vi "Tutorial.vi"() -> ()   [LabVIEW 2026]
uses:
  C:/Users/loicw/Documents/LabVIEW/ToastNotifications/Sources/bins/Microsoft.Toolkit.Uwp.Notifications.dll
  bins/Microsoft.Toolkit.Uwp.Notifications.dll
panel:
  out "GetContent":string
  out "Arguments":string
  out "WasCurrentProcessToastActivated":bool
  in  "stop":bool
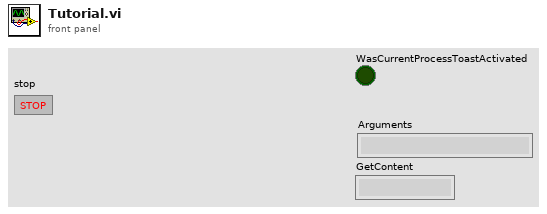
[diagram p1: front panel]
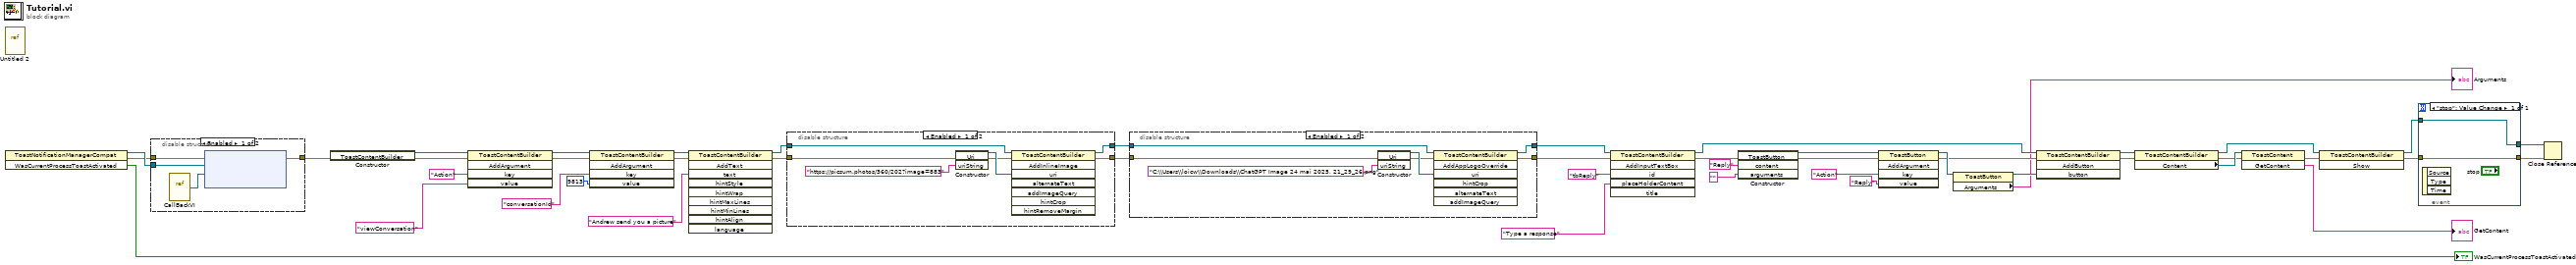
[diagram p0: block diagram]
diagram:
  n1 = vi-ref "Untitled 2.vi"() -> ()  [unwired: 1 out]
  n2 = invoke class="ToastNotificationManagerCompat" method="WasCurrentProcessToastActivated"() -> (reference out=w17:refnum<k24>, error out=w16:errorcluster, "WasCurrentProcessToastActivated"=→"WasCurrentProcessToastActivated":bool)  [unwired: 3 in]
  n3 = disable-structure shown="Enabled" {
    disable-tunnel: w17 -> [w50 _]
    disable-tunnel: w16 -> [w49 w51]
    disable-tunnel: [w48 w51] -> w15
    frame Enabled {
      n4 = vi-ref "CallBackVI.vi"() -> ("vi reference"=w47:refnum<vi>)
      n5 = node(w49, w50, w47) -> (w48:errorcluster)  [unwired: 2 in, 1 out]
    }
    frame Disabled {
    }
  }
  n6 = constructor class="ToastContentBuilder"(error in=w15) -> (reference out=w45:refnum<k24>, error out=w46:errorcluster)  [unwired: 2 in, 1 out]
  n7 = invoke class="ToastContentBuilder" method="AddArgument"(reference=w45, error in=w46, "key"="Action", "value"="viewConversation") -> (reference out=w42:refnum<k24>, error out=w41:errorcluster)  [unwired: 1 in, 3 out]
  n8 = invoke class="ToastContentBuilder" method="AddArgument"(reference=w42, error in=w41, "key"="conversationId", "value"=9813) -> (reference out=w38:refnum<k24>, error out=w37:errorcluster)  [unwired: 1 in, 3 out]
  n9 = invoke class="ToastContentBuilder" method="AddText"(reference=w38, error in=w37, "text"="Andrew send you a picture") -> (reference out=w31:refnum<k24>, error out=w13:errorcluster)  [unwired: 7 in, 8 out]
  n10 = disable-structure shown="Enabled" {
    disable-tunnel: w31 -> [w58 w60]
    disable-tunnel: [w55 w60] -> w30
    disable-tunnel: w13 -> [w54 w59]
    disable-tunnel: [w52 w59] -> w12
    frame Enabled {
      n11 = constructor class="Uri"(error in=w54, "uriString"="https://picsum.photos/360/202?image=883") -> (reference out=w57:refnum<k24>, error out=w53:errorcluster)  [unwired: 2 in, 2 out]
      n12 = invoke class="ToastContentBuilder" method="AddInlineImage"(reference=w58, error in=w53, "uri"=w57) -> (reference out=w55:refnum<k24>, error out=w52:errorcluster)  [unwired: 5 in, 6 out]
    }
    frame Disabled {
    }
  }
  n13 = disable-structure shown="Enabled" {
    disable-tunnel: w30 -> [w67 w68]
    disable-tunnel: [w64 w69] -> w29
    disable-tunnel: [w63 w68] -> w28
    disable-tunnel: w12 -> [w62 w69]
    frame Enabled {
      n14 = constructor class="Uri"(error in=w62, "uriString"="C:\\Users\\loicw\\Downloads\\ChatGPT Image 24 mai 2025, 21_29_26.png") -> (reference out=w66:refnum<k24>, error out=w61:errorcluster)  [unwired: 2 in, 2 out]
      n15 = invoke class="ToastContentBuilder" method="AddAppLogoOverride"(reference=w67, error in=w61, "uri"=w66) -> (reference out=w63:refnum<k24>, error out=w64:errorcluster)  [unwired: 4 in, 5 out]
    }
    frame Disabled {
    }
  }
  n16 = invoke class="ToastContentBuilder" method="AddInputTextBox"(reference=w28, error in=w29, "id"="tbReply", "placeHolderContent"="Type a response") -> (reference out=w20:refnum<k24>, error out=w10:errorcluster)  [unwired: 2 in, 4 out]
  n17 = constructor class="ToastButton"(error in=w10, "content"="Reply", "arguments"="") -> (reference out=w21:refnum<k24>, error out=w11:errorcluster)  [unwired: 2 in, 3 out]
  n18 = invoke class="ToastButton" method="AddArgument"(reference=w21, error in=w11, "key"="Action", "value"="Reply") -> (reference out=w18:refnum<k24>, error out=w9:errorcluster)  [unwired: 1 in, 3 out]
  n19 = property class="ToastButton"(reference=w18) -> (reference out=w8:refnum<k24>, "Arguments"=→"Arguments":string)  [unwired: 1 in, 1 out]
  n20 = invoke class="ToastContentBuilder" method="AddButton"(reference=w20, error in=w9, "button"=w8) -> (reference out=w19:refnum<k24>, error out=w5:errorcluster)  [unwired: 1 in, 2 out]
  n21 = property class="ToastContentBuilder"(reference=w19, error in=w5) -> (reference out=w6:refnum<k24>, error out=w3:errorcluster, "Content"=w4:refnum<k24>)
  n22 = invoke class="ToastContent" method="GetContent"(reference=w4, error in=w3) -> (error out=w2:errorcluster, "GetContent"=→"GetContent":string)  [unwired: 1 in, 1 out]
  n23 = invoke class="ToastContentBuilder" method="Show"(reference=w6, error in=w2) -> (reference out=w34:refnum<k24>, error out=w35:errorcluster)  [unwired: 1 in, 1 out]
  n24 = event shown="[0] \"stop\": Value Change" {
    selector: _ -> [_]
    dyn-events: _ -> [_]
    timeout: _ -> [_]
    tunnel: w35 -> [w70]
    tunnel: w34 -> [w71]
    tunnel: [w71] -> w32
    tunnel: [w70] -> w33
    event "stop": Value Change {
      n25 = event-data() -> ()  [unwired: 1 in, 3 out]
    }
  }
  n26 = Close Reference(reference=w32, error in (no error)=w33) -> ()  [unwired: 1 out]
